vi "TCP Connect.vi"(9 "端口":u16, 10 "Sever IP":string, 11 "终端":enum16{"Server", "Client"}(ring)) -> (2 "TCP网络连接输出":refnum<k5>, 3 "Connection Status":T1)   [LabVIEW 2020, in "TCP Communication.lvlib"]
uses:
  TCP Communication.lvlib
  Connection Status.ctl
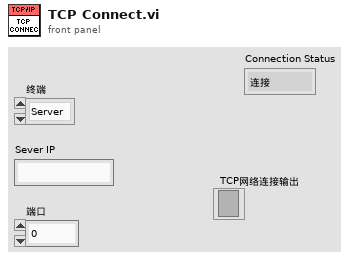
[diagram p1: front panel]
types:
  T1 = typedef "TCP Communication.lvlib/Connection Status.ctl" = enum16{"连接", "通信", "关闭"}
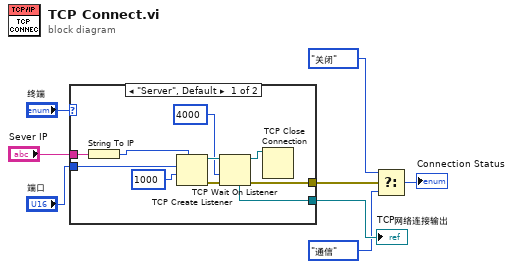
[diagram p0: block diagram]
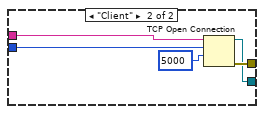
[diagram p2: hidden frame]
diagram:
  n1 = case shown="\"Server\", Default" "终端" {
    tunnel: "端口" -> [w18 w23]
    tunnel: [w17 w19] -> w6
    tunnel: [w16 w20] -> w4
    tunnel: "Sever IP" -> [w10 w22]
    frame "Server", Default {
      n2 = String To IP(1:w10) -> (0:w9:u32)
      n3 = TCP Create Listener(7:w9, 9:1000 ("超时毫秒(25000)"), 10:w18) -> (0:w14:errorcluster, 3:w15:refnum<k5>)  [unwired: 2 in, 1 out]
      n4 = TCP Wait On Listener(8:w14, 9:4000 ("超时毫秒(25000)"), 11:w15) -> (0:w16:errorcluster, 3:w11:refnum<k5>, 4:w17:refnum<k5>)  [unwired: 1 in, 2 out]
      n5 = TCP Close Connection(connection ID=w11) -> ()  [unwired: 2 in, 2 out]
    }
    frame "Client" {
      n6 = TCP Open Connection(address=w22, remote port or service name=w23, timeout ms (60000)=5000 ("超时毫秒(60000)")) -> (connection ID=w19:refnum<k5>, error out=w20:errorcluster)  [unwired: 2 in]
    }
  }
  "TCP网络连接输出" <- w6
  n7 = Select(t=Connection_Status."关闭" ("连接状态"), s=w4, f=Connection_Status."通信" ("连接状态")) -> (s? t:f=→"Connection Status":T1)
